vi "Read Ex.vi"(8 "error in (no error)":errorcluster, 9 "LARGO":u32, 10 "PID":u32, 11 "VID":u32) -> (0 "error out":errorcluster, 1 "DATOS":u8[](array[numeric]), 3 "OUT":i32)   [LabVIEW 2011, in "HID_ARZ.lvlib"]
doc: "READ_EX ReadEx;"
uses:
  HID_ARZ.lvlib
  <userlib>/HID_ARZ/mcHID.dll
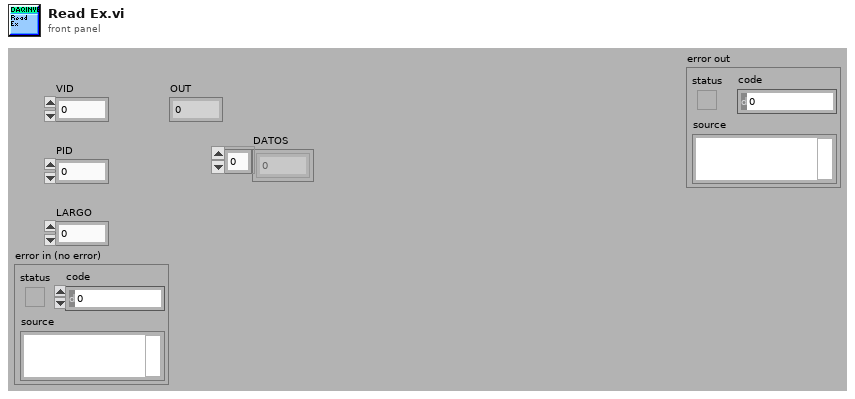
[diagram p1: front panel]
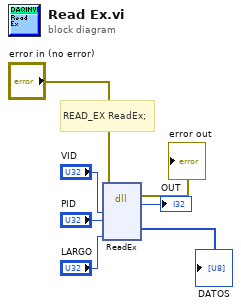
[diagram p0: block diagram]
diagram:
  # "READ_EX ReadEx;"
  n1 = dll-call lib="C:/Program Files (x86)/National Instruments/LabVIEW 2017/user.lib/HID_ARZ/mcHID.*" fn="ReadEx"(error in="error in (no error)", "VID"="VID", "PID"="PID", "LARGO"="LARGO") -> (error out=→"error out":errorcluster, "return type"=→"OUT":i32, "DATOS"=→"DATOS":u8[])  [unwired: 6 in, 1 out]
